vi "02_ui_plot_window.vi"() -> ()   [LabVIEW 2025]
uses:
  4c7a61b9-d50a-4fa5-8b88-644507a3af04.vi
  74ea501e-f43b-483f-8511-84a735437533.vi
  166e0385-1291-4ee6-a608-8b02bdaae3d2.vi
  b1158e5f-e22e-42fa-9d41-9ea4e4d0b9e3.vi
  31b119fa-27fe-4ebe-809c-2da1a8fd4d96.vi
  13143f16-a64c-4a8d-9511-2945b8db9dc5.vi
  9c1d92a2-1c85-4809-97a6-d36bf52cbad7.vi
  d684625a-03c4-4daf-8e9e-674a236ebb3e.vi
  fb960f78-e1fe-4b5d-8417-6d8be925c5cf.vi
  c135c75a-78bf-4448-8d92-d4bbbd51cd11.vi
  <vilib>/Utility/config.llb/Read Key (U32).vi
  <vilib>/Utility/config.llb/Read Key (Boolean).vi
  <vilib>/Utility/config.llb/Read Key (String).vi
  <vilib>/Utility/config.llb/Write Key (U32).vi
  <vilib>/Utility/config.llb/Write Key (Boolean).vi
  <vilib>/Utility/config.llb/Write Key (String).vi
  00_global_variables.vi
  <vilib>/Utility/config.llb/NI_LVConfig.lvlib
panel:
  out "loaded_config_path":path
  out "loaded_config_filename":string caption="Recent File"
  in  "open_config_plot_0":bool
  in  "safe_config_as_plot_0":bool
  in  "safe_config_plot_0":bool
  in  "select_plot_5":string(combo)="2"
  in  "select_plot_4":string(combo)="2"
  out "cursor_p5_1_prefix":string
  out "cursor_p4_1_prefix":string
  out "cursor_p5_2_prefix":string
  out "cursor_p4_2_prefix":string
  out "cursor_p5_2":dbl format="%#_6f"
  in  "color_picker_5":u32(colorbox)=14811391
  out "cursor_p5_1":dbl format="%#_6f"
  in  "enable_plot_5":bool caption="S11 - Imaginary"
  out "cursor_p4_2":dbl format="%#_6f"
  in  "color_picker_4":u32(colorbox)=49352
  out "cursor_p4_1":dbl format="%#_6f"
  in  "enable_plot_4":bool caption="S11 - Imaginary"
  in  "select_plot_3":string(combo)="2"
  in  "select_plot_2":string(combo)="2"
  in  "select_plot_1":string(combo)="2"
  in  "select_plot_0":string(combo)="2"
  out "cursor_p3_1_prefix":string
  out "cursor_p2_1_prefix":string
  out "cursor_p1_1_prefix":string
  out "cursor_p0_1_prefix":string
  out "cursor_p3_2_prefix":string
  out "cursor_p2_2_prefix":string
  out "cursor_p1_2_prefix":string
  out "cursor_p0_2_prefix":string
  out "cursor_p3_2":dbl format="%#_6f"
  in  "color_picker_3":u32(colorbox)=14468608
  out "cursor_p3_1":dbl format="%#_6f"
  in  "enable_plot_3":bool caption="S11 - Imaginary"
  out "cursor_p2_2":dbl format="%#_6f"
  in  "color_picker_2":u32(colorbox)=39219
  out "cursor_p2_1":dbl format="%#_6f"
  in  "enable_plot_2":bool caption="S11 - Imaginary"
  out "cursor_p1_2":dbl format="%#_6f"
  out "cursor_p0_2":dbl format="%#_6f"
  out "cursor_p0_freq_2":string caption="Frequenz"
  out "cursor_p0_wavel_2":dbl caption="Frequenz"
  out "cursor_p0_wavel_1":dbl caption="Frequenz"
  in  "color_picker_1":u32(colorbox)=14423100
  in  "color_picker_0":u32(colorbox)=26316
  out "cursor_p0_freq_1":string caption="Frequenz"
  out "cursor_p1_1":dbl format="%#_6f"
  out "cursor_p0_1":dbl format="%#_6f"
  in  "enable_plot_1":bool caption="S11 - Imaginary"
  in  "enable_plot_0":bool=TRUE
  out "plot_0":cluster{"array type (2D Dbl)":dbl[], dbl[]}[](graph)
  # "Cursor 2"
  # "Cursor 1"
  # "Hz"
  # "Frequency"
  # "Hz"
  # "Wavelength"
  # "m"
  # "m"
  # "Configuration"
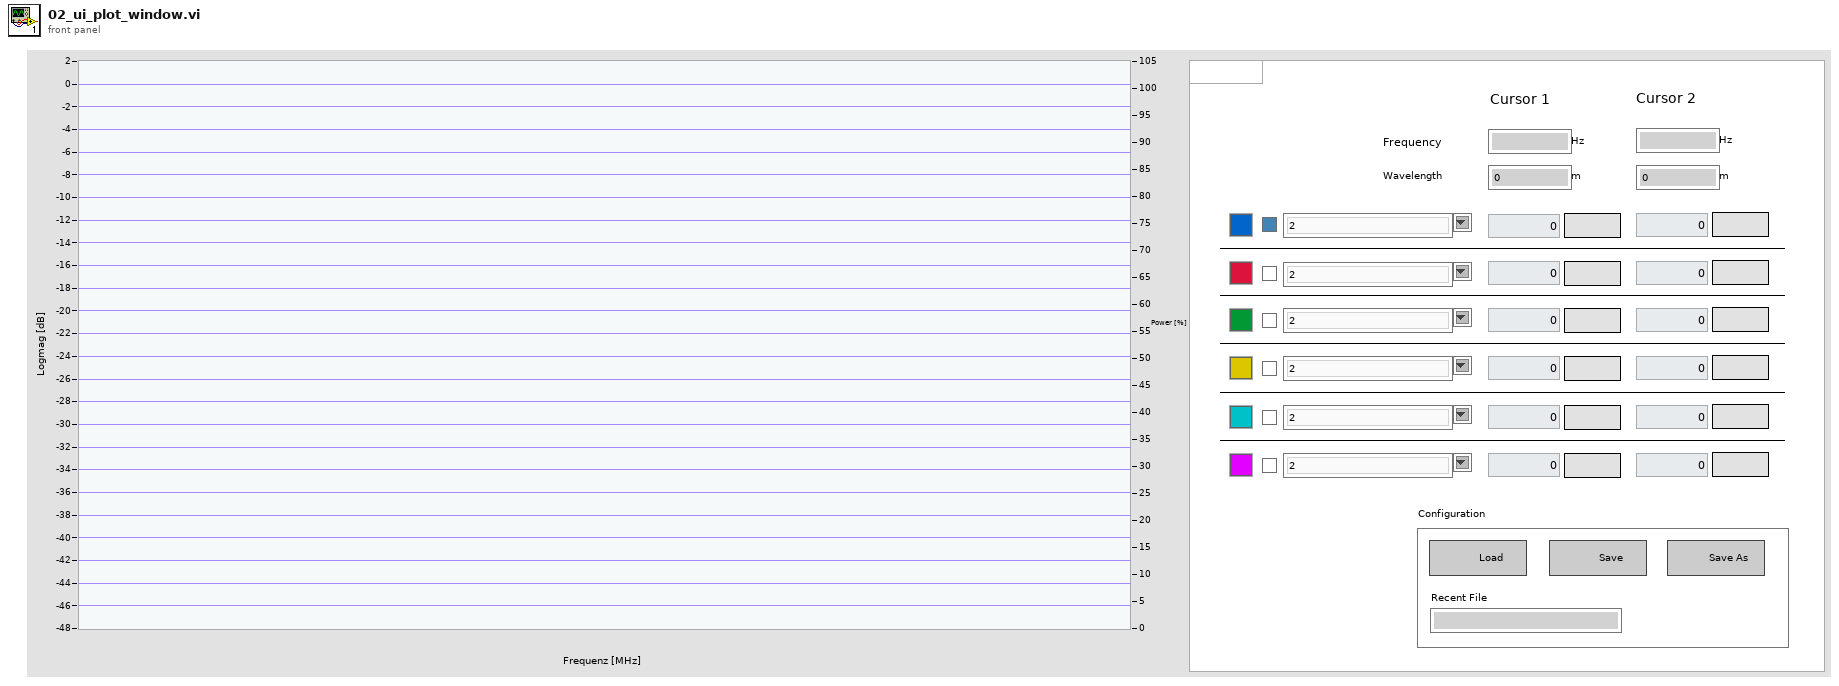
[diagram p1: front panel]
types:
  T1 = typedef "NI_LVConfig.lvlib/Config Data RefNum.ctl" = refnum<k1>
  T2 = typedef "LVComboBoxStrsAndValuesArrayTypeDef.ctl" = cluster{"String":string, "Value":string}[]
  T3 = cluster{"freq_array":dbl[], "data_array":dbl[]}[]
  T4 = cluster{"y_scale_id":u32, "unit":string, "prefix_enable":bool, "plot_id":u32}[]
  T5 = cluster{"y_scale_id":u32, "unit":string, "prefix_enable":bool, "plot_id":u32}
  T6 = typedef "LVCursorListTypeDef.ctl" = cluster{"Name":string, "Color":u32, "Style":u8, "Point Style":u8, "Name Visible":bool, "Allow Drag":bool, "Cursor Mode":u32, "Plot":i32, "Index":i32, "Position":cluster{"X":dbl, "Y":dbl}, "X Scale":u32, "Y Scale":u32, "Watch Plots":i32[], "Watch All Plots":bool, "Plot Area":i32, "Label Offset":cluster{"X":dbl, "Y":dbl}}[]
  T7 = cluster{"cursor_data":dbl[], "frequency":string, "wavelength_m":dbl}
  T8 = cluster{"cursor_0_color":u32, "cursor_1_color":u32}
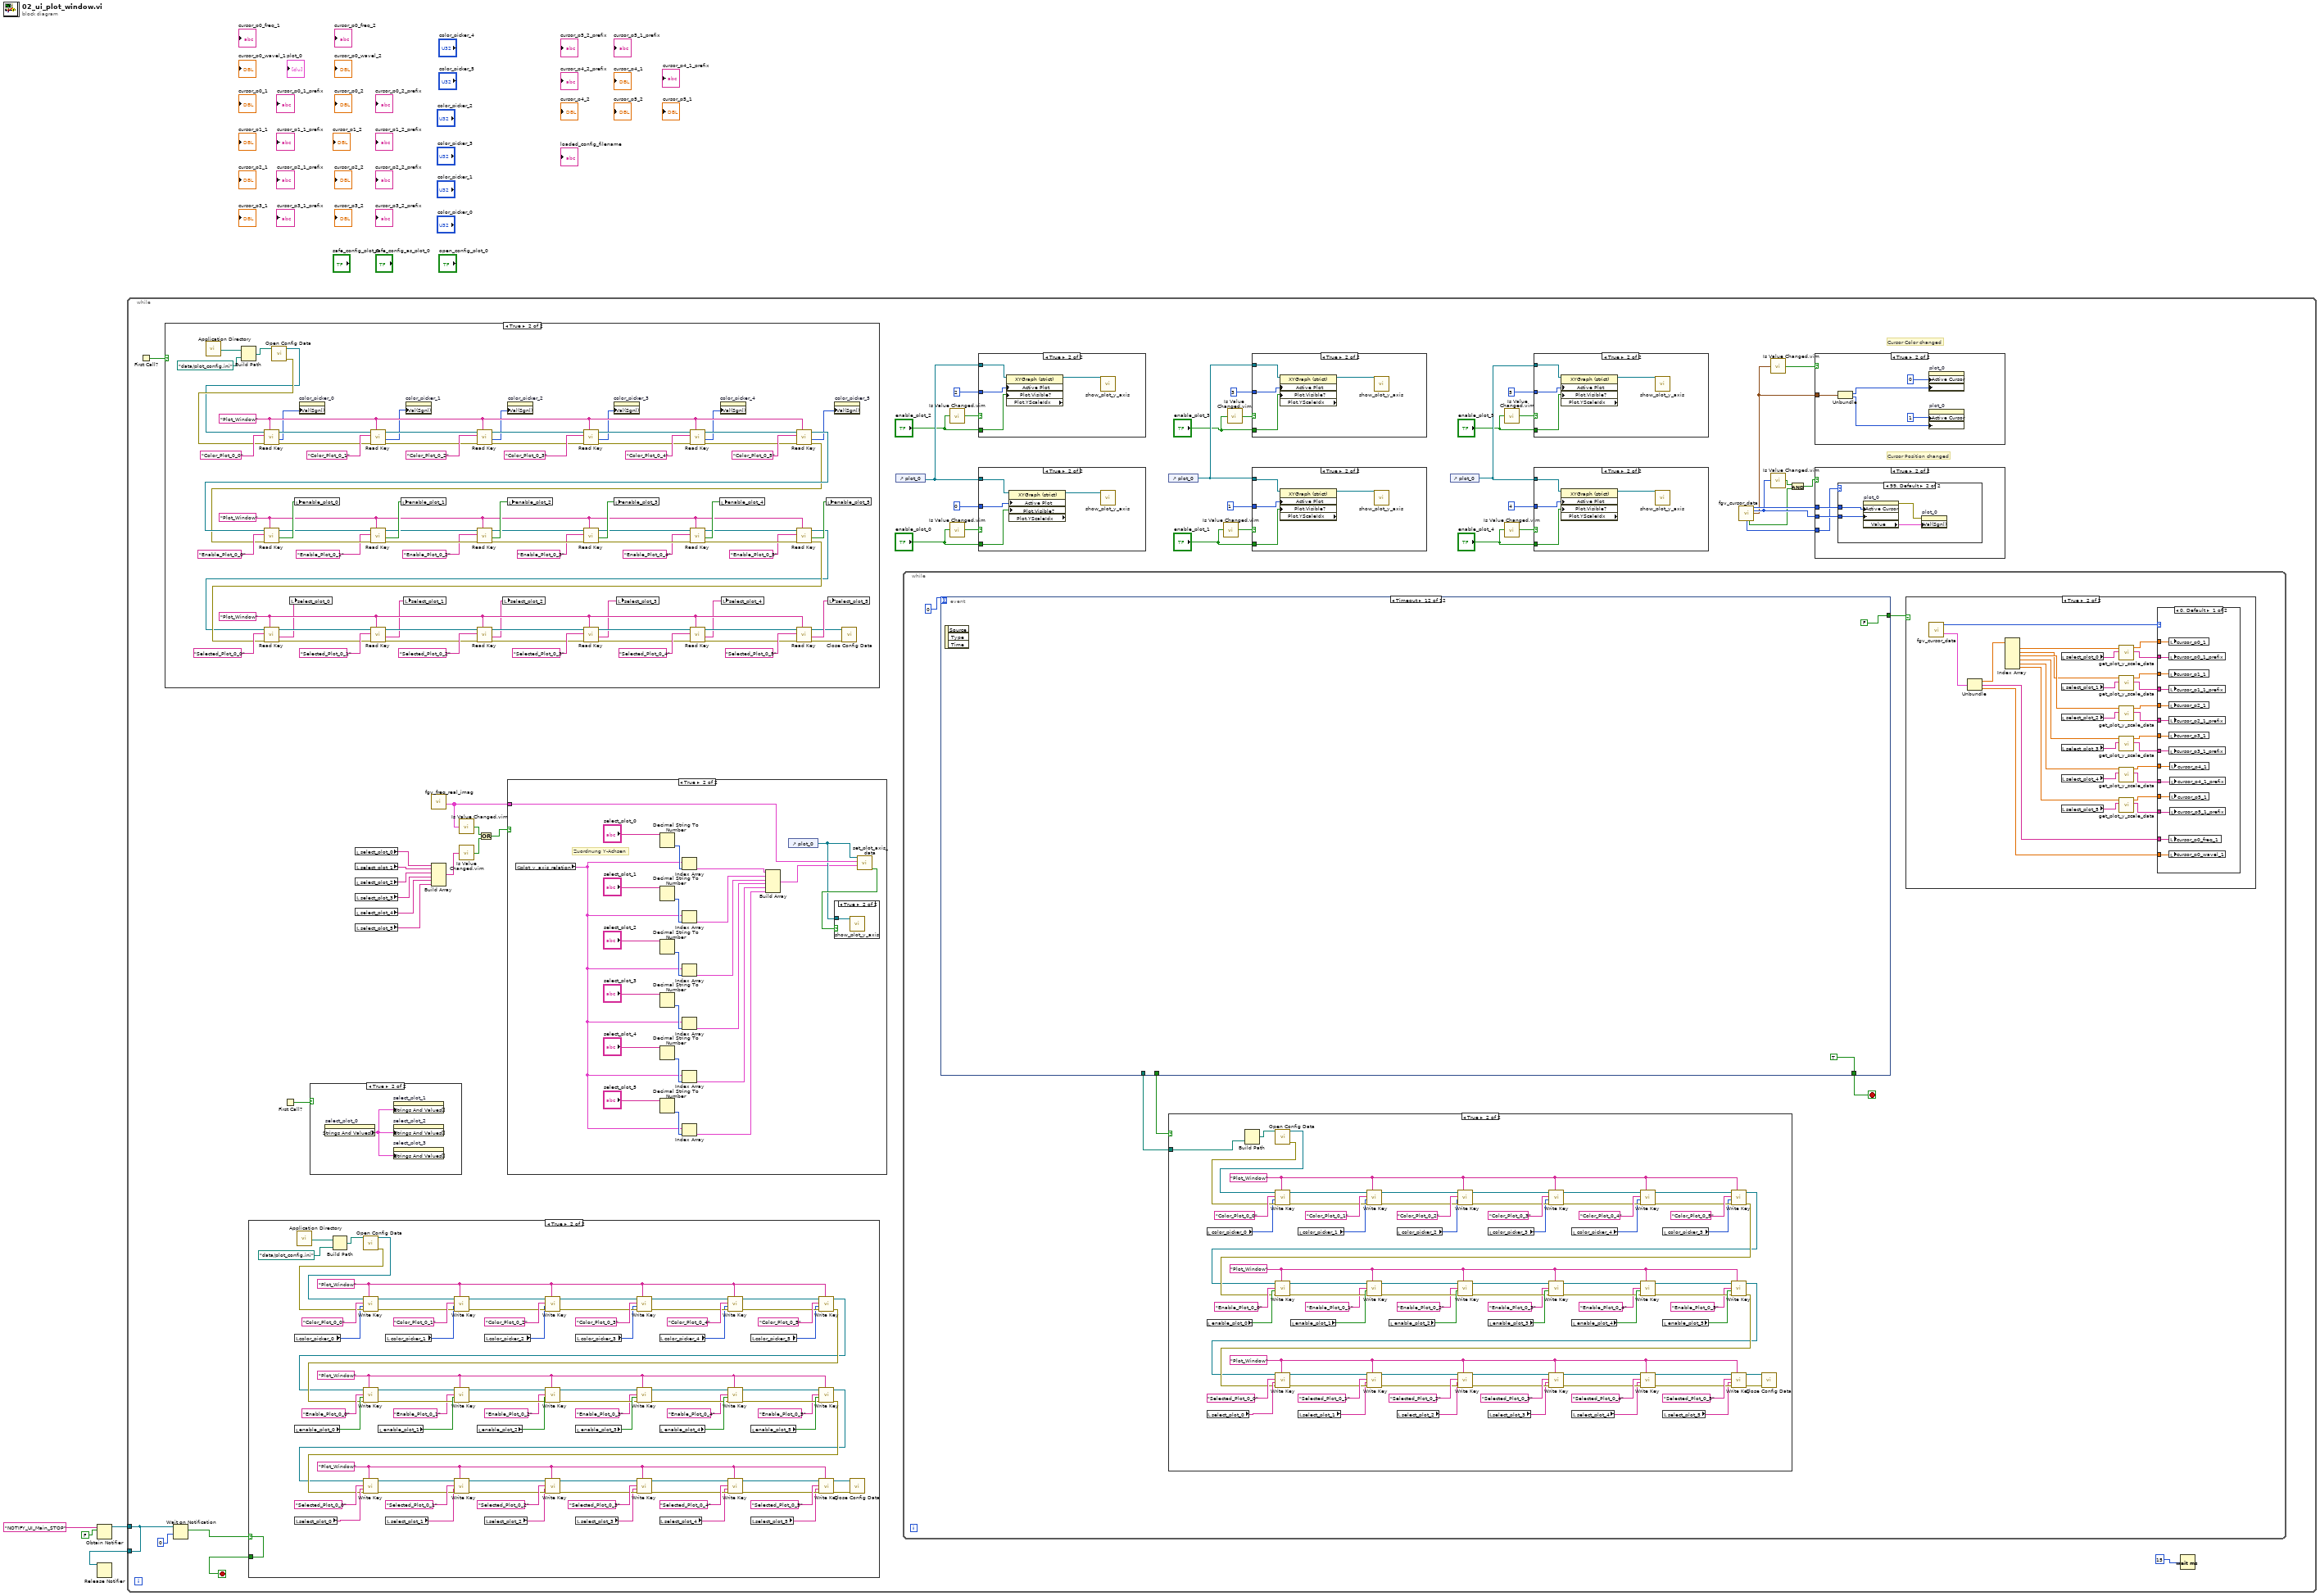
[diagram p0: block diagram]
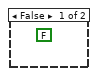
[diagram p11: hidden frame]
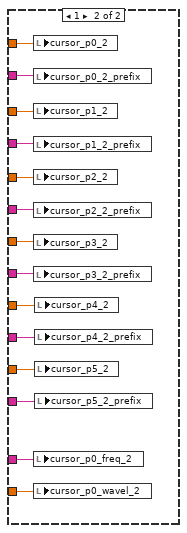
[diagram p18: hidden frame]
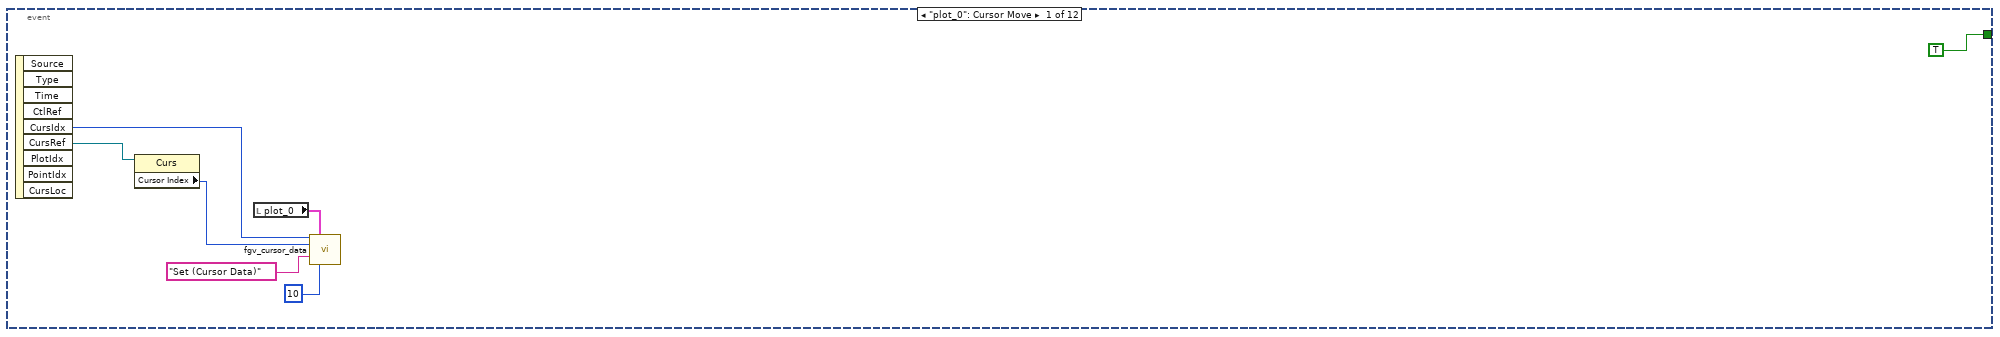
[diagram p19: hidden frame]
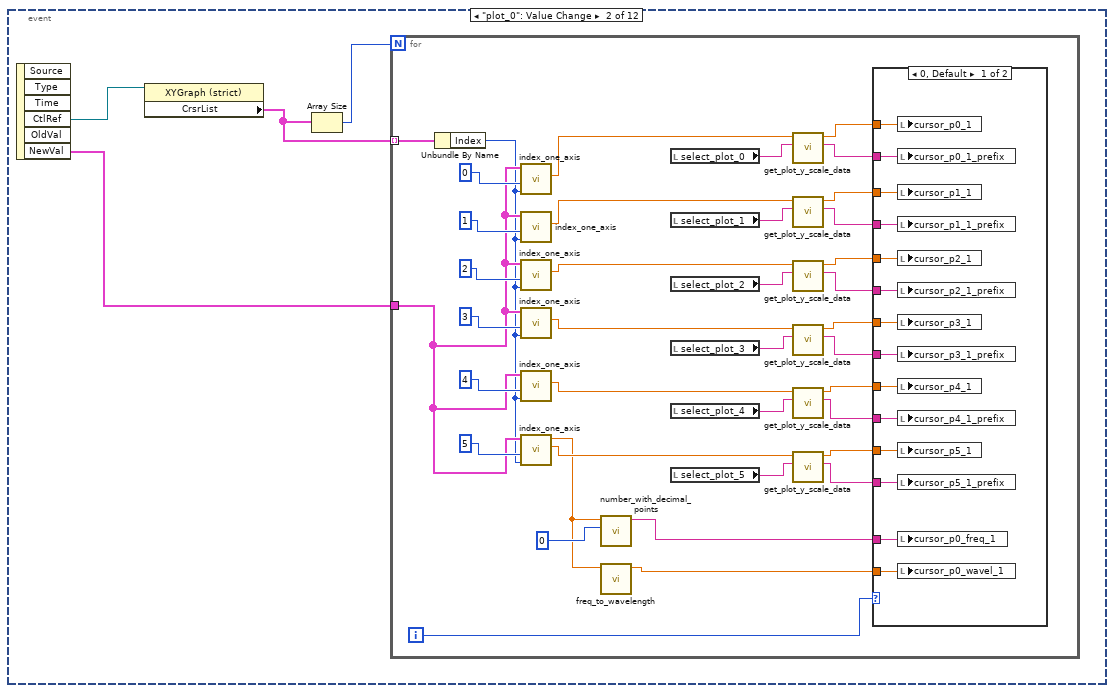
[diagram p20: hidden frame]
diagram:
  n1 = Obtain Notifier(name (unnamed)="NOTIFY_UI_Main_STOP", notification data type=FALSE) -> (notifier out=w2:refnum<notifier>)  [unwired: 2 in, 2 out]
  n2 = while {
    tunnel: w2 -> [w28]
    tunnel: [w28] -> w1
    stop <- w14 stop-if-true
    # "Cursor Color changed"
    # "Cursor Position changed"
    n3 = First Call?() -> (First Call?: T/F=w13:bool)
    n4 = case shown="True" w13 {
      frame False {
      }
      frame True {
        w166 = "Plot_Window" ("section")
        w201 = "Plot_Window" ("section")
        w208 = "Plot_Window" ("section")
        n5 = call <vilib>:"Application Directory.vi"() -> ("Application Directory"=w151:path)
        n6 = Build Path(base path=w151, name or relative path=path "data/plot_config.ini") -> (appended path=w157:path)
        n7 = call <vilib>:"Open Config Data.vi"("configuration file path"=w157) -> ("error out"=w155:errorcluster, "refnum"=w154:T1)  [unwired: 8 in, 1 out]
        n8 = call-poly <vilib>:"Read Key.vi"("section"=w208, "error in (no error)"=w155, "key"="Color_Plot_0_0", "refnum"=w154) -> ("error out"=w221:errorcluster, "value"=w150:u32, "refnum out"=w222:T1)  [unwired: 4 in, 1 out]
        n9 = property on="color_picker_0" class="ColBox"("Val(Sgnl)"=w150) -> ()  [unwired: 2 in, 2 out]
        n10 = call-poly <vilib>:"Read Key.vi"("section"=w208, "error in (no error)"=w221, "key"="Color_Plot_0_1", "refnum"=w222) -> ("error out"=w218:errorcluster, "value"=w149:u32, "refnum out"=w219:T1)  [unwired: 4 in, 1 out]
        n11 = property on="color_picker_1" class="ColBox"("Val(Sgnl)"=w149) -> ()  [unwired: 2 in, 2 out]
        n12 = call-poly <vilib>:"Read Key.vi"("section"=w208, "error in (no error)"=w218, "key"="Color_Plot_0_2", "refnum"=w219) -> ("error out"=w215:errorcluster, "value"=w145:u32, "refnum out"=w216:T1)  [unwired: 4 in, 1 out]
        n13 = property on="color_picker_2" class="ColBox"("Val(Sgnl)"=w145) -> ()  [unwired: 2 in, 2 out]
        n14 = call-poly <vilib>:"Read Key.vi"("section"=w208, "error in (no error)"=w215, "key"="Color_Plot_0_3", "refnum"=w216) -> ("error out"=w212:errorcluster, "value"=w146:u32, "refnum out"=w213:T1)  [unwired: 4 in, 1 out]
        n15 = property on="color_picker_3" class="ColBox"("Val(Sgnl)"=w146) -> ()  [unwired: 2 in, 2 out]
        n16 = call-poly <vilib>:"Read Key.vi"("section"=w208, "error in (no error)"=w212, "key"="Color_Plot_0_4", "refnum"=w213) -> ("error out"=w210:errorcluster, "value"=w147:u32, "refnum out"=w209:T1)  [unwired: 4 in, 1 out]
        n17 = property on="color_picker_4" class="ColBox"("Val(Sgnl)"=w147) -> ()  [unwired: 2 in, 2 out]
        n18 = call-poly <vilib>:"Read Key.vi"("section"=w208, "error in (no error)"=w210, "key"="Color_Plot_0_5", "refnum"=w209) -> ("error out"=w183:errorcluster, "value"=w148:u32, "refnum out"=w184:T1)  [unwired: 4 in, 1 out]
        n19 = call-poly <vilib>:"Read Key.vi"("section"=w201, "error in (no error)"=w183, "key"="Enable_Plot_0_0", "refnum"=w184) -> ("error out"=w188:errorcluster, "value"=w202:bool, "refnum out"=w187:T1)  [unwired: 4 in, 1 out]
        n20 = local write "enable_plot_0"(w202) -> ()
        n21 = call-poly <vilib>:"Read Key.vi"("section"=w201, "error in (no error)"=w188, "key"="Enable_Plot_0_1", "refnum"=w187) -> ("error out"=w191:errorcluster, "value"=w203:bool, "refnum out"=w190:T1)  [unwired: 4 in, 1 out]
        n22 = local write "enable_plot_1"(w203) -> ()
        n23 = call-poly <vilib>:"Read Key.vi"("section"=w201, "error in (no error)"=w191, "key"="Enable_Plot_0_2", "refnum"=w190) -> ("error out"=w194:errorcluster, "value"=w204:bool, "refnum out"=w193:T1)  [unwired: 4 in, 1 out]
        n24 = local write "enable_plot_2"(w204) -> ()
        n25 = call-poly <vilib>:"Read Key.vi"("section"=w201, "error in (no error)"=w194, "key"="Enable_Plot_0_3", "refnum"=w193) -> ("error out"=w197:errorcluster, "value"=w205:bool, "refnum out"=w196:T1)  [unwired: 4 in, 1 out]
        n26 = local write "enable_plot_3"(w205) -> ()
        n27 = call-poly <vilib>:"Read Key.vi"("section"=w201, "error in (no error)"=w197, "key"="Enable_Plot_0_4", "refnum"=w196) -> ("error out"=w199:errorcluster, "value"=w206:bool, "refnum out"=w200:T1)  [unwired: 4 in, 1 out]
        n28 = local write "enable_plot_4"(w206) -> ()
        n29 = call-poly <vilib>:"Read Key.vi"("section"=w201, "error in (no error)"=w199, "key"="Enable_Plot_0_5", "refnum"=w200) -> ("error out"=w159:errorcluster, "value"=w207:bool, "refnum out"=w158:T1)  [unwired: 4 in, 1 out]
        n30 = call-poly <vilib>:"Read Key.vi"("section"=w166, "error in (no error)"=w159, "key"="Selected_Plot_0_0", "refnum"=w158) -> ("error out"=w179:errorcluster, "value"=w165:string, "refnum out"=w180:T1)  [unwired: 4 in, 1 out]
        n31 = local write "select_plot_0"(w165) -> ()
        n32 = call-poly <vilib>:"Read Key.vi"("section"=w166, "error in (no error)"=w179, "key"="Selected_Plot_0_1", "refnum"=w180) -> ("error out"=w176:errorcluster, "value"=w164:string, "refnum out"=w177:T1)  [unwired: 4 in, 1 out]
        n33 = local write "select_plot_1"(w164) -> ()
        n34 = call-poly <vilib>:"Read Key.vi"("section"=w166, "error in (no error)"=w176, "key"="Selected_Plot_0_2", "refnum"=w177) -> ("error out"=w173:errorcluster, "value"=w163:string, "refnum out"=w174:T1)  [unwired: 4 in, 1 out]
        n35 = local write "select_plot_2"(w163) -> ()
        n36 = call-poly <vilib>:"Read Key.vi"("section"=w166, "error in (no error)"=w173, "key"="Selected_Plot_0_3", "refnum"=w174) -> ("error out"=w170:errorcluster, "value"=w162:string, "refnum out"=w171:T1)  [unwired: 4 in, 1 out]
        n37 = local write "select_plot_3"(w162) -> ()
        n38 = call-poly <vilib>:"Read Key.vi"("section"=w166, "error in (no error)"=w170, "key"="Selected_Plot_0_4", "refnum"=w171) -> ("error out"=w168:errorcluster, "value"=w161:string, "refnum out"=w167:T1)  [unwired: 4 in, 1 out]
        n39 = local write "select_plot_4"(w161) -> ()
        n40 = call-poly <vilib>:"Read Key.vi"("section"=w166, "error in (no error)"=w168, "key"="Selected_Plot_0_5", "refnum"=w167) -> ("error out"=w152:errorcluster, "value"=w160:string, "refnum out"=w153:T1)  [unwired: 4 in, 1 out]
        n41 = local write "enable_plot_5"(w207) -> ()
        n42 = local write "select_plot_5"(w160) -> ()
        n43 = property on="color_picker_5" class="ColBox"("Val(Sgnl)"=w148) -> ()  [unwired: 2 in, 2 out]
        n44 = call <vilib>:"Close Config Data.vi"("error in (no error)"=w152, "refnum"=w153) -> ()  [unwired: 8 in, 2 out]
      }
    }
    n45 = Wait on Notification(notifier=w28, timeout in ms (-1)=0) -> (notification=w15:bool)  [unwired: 2 in, 3 out]
    n46 = case shown="True" w15 {
      selector: w15 -> [_ w144]
      tunnel: [_ w144] -> w14
      frame False {
      }
      frame True {
        w71 = "Plot_Window" ("section")
        w116 = "Plot_Window" ("section")
        w65 = "Plot_Window" ("section")
        n47 = local read "color_picker_0"() -> (w123:u32)
        n48 = local read "enable_plot_0"() -> (w111:bool)
        n49 = local read "select_plot_0"() -> (w76:string)
        n50 = call <vilib>:"Application Directory.vi"() -> ("Application Directory"=w64:path)
        n51 = Build Path(base path=w64, name or relative path=path "data/plot_config.ini") -> (appended path=w130:path)
        n52 = call <vilib>:"Open Config Data.vi"("configuration file path"=w130) -> ("error out"=w128:errorcluster, "refnum"=w127:T1)  [unwired: 8 in, 1 out]
        n53 = call-poly <vilib>:"Write Key.vi"("section"=w65, "error in (no error)"=w128, "value"=w123, "key"="Color_Plot_0_0", "refnum"=w127) -> ("error out"=w140:errorcluster, "refnum out"=w141:T1)  [unwired: 4 in, 1 out]
        n54 = local read "enable_plot_1"() -> (w112:bool)
        n55 = local read "color_picker_1"() -> (w122:u32)
        n56 = local read "select_plot_1"() -> (w75:string)
        n57 = call-poly <vilib>:"Write Key.vi"("section"=w65, "error in (no error)"=w140, "value"=w122, "key"="Color_Plot_0_1", "refnum"=w141) -> ("error out"=w137:errorcluster, "refnum out"=w138:T1)  [unwired: 4 in, 1 out]
        n58 = local read "enable_plot_2"() -> (w113:bool)
        n59 = local read "color_picker_2"() -> (w121:u32)
        n60 = local read "select_plot_2"() -> (w74:string)
        n61 = call-poly <vilib>:"Write Key.vi"("section"=w65, "error in (no error)"=w137, "value"=w121, "key"="Color_Plot_0_2", "refnum"=w138) -> ("error out"=w134:errorcluster, "refnum out"=w135:T1)  [unwired: 4 in, 1 out]
        n62 = local read "color_picker_3"() -> (w118:u32)
        n63 = local read "enable_plot_3"() -> (w117:bool)
        n64 = local read "select_plot_3"() -> (w70:string)
        n65 = call-poly <vilib>:"Write Key.vi"("section"=w65, "error in (no error)"=w134, "value"=w118, "key"="Color_Plot_0_3", "refnum"=w135) -> ("error out"=w131:errorcluster, "refnum out"=w132:T1)  [unwired: 4 in, 1 out]
        n66 = local read "color_picker_4"() -> (w120:u32)
        n67 = local read "enable_plot_4"() -> (w114:bool)
        n68 = local read "select_plot_4"() -> (w73:string)
        n69 = call-poly <vilib>:"Write Key.vi"("section"=w65, "error in (no error)"=w131, "value"=w120, "key"="Color_Plot_0_4", "refnum"=w132) -> ("error out"=w124:errorcluster, "refnum out"=w125:T1)  [unwired: 4 in, 1 out]
        n70 = local read "color_picker_5"() -> (w119:u32)
        n71 = local read "enable_plot_5"() -> (w115:bool)
        n72 = local read "select_plot_5"() -> (w72:string)
        n73 = call-poly <vilib>:"Write Key.vi"("section"=w65, "error in (no error)"=w124, "value"=w119, "key"="Color_Plot_0_5", "refnum"=w125) -> ("error out"=w94:errorcluster, "refnum out"=w93:T1)  [unwired: 4 in, 1 out]
        n74 = call-poly <vilib>:"Write Key.vi"("section"=w116, "error in (no error)"=w94, "value"=w111, "key"="Enable_Plot_0_0", "refnum"=w93) -> ("error out"=w98:errorcluster, "refnum out"=w97:T1)  [unwired: 4 in, 1 out]
        n75 = call-poly <vilib>:"Write Key.vi"("section"=w116, "error in (no error)"=w98, "value"=w112, "key"="Enable_Plot_0_1", "refnum"=w97) -> ("error out"=w101:errorcluster, "refnum out"=w100:T1)  [unwired: 4 in, 1 out]
        n76 = call-poly <vilib>:"Write Key.vi"("section"=w116, "error in (no error)"=w101, "value"=w113, "key"="Enable_Plot_0_2", "refnum"=w100) -> ("error out"=w104:errorcluster, "refnum out"=w103:T1)  [unwired: 4 in, 1 out]
        n77 = call-poly <vilib>:"Write Key.vi"("section"=w116, "error in (no error)"=w104, "value"=w117, "key"="Enable_Plot_0_3", "refnum"=w103) -> ("error out"=w107:errorcluster, "refnum out"=w106:T1)  [unwired: 4 in, 1 out]
        n78 = call-poly <vilib>:"Write Key.vi"("section"=w116, "error in (no error)"=w107, "value"=w114, "key"="Enable_Plot_0_4", "refnum"=w106) -> ("error out"=w110:errorcluster, "refnum out"=w109:T1)  [unwired: 4 in, 1 out]
        n79 = call-poly <vilib>:"Write Key.vi"("section"=w116, "error in (no error)"=w110, "value"=w115, "key"="Enable_Plot_0_5", "refnum"=w109) -> ("error out"=w69:errorcluster, "refnum out"=w68:T1)  [unwired: 4 in, 1 out]
        n80 = call-poly <vilib>:"Write Key.vi"("section"=w71, "error in (no error)"=w69, "value"=w76, "key"="Selected_Plot_0_0", "refnum"=w68) -> ("error out"=w89:errorcluster, "refnum out"=w90:T1)  [unwired: 4 in, 1 out]
        n81 = call-poly <vilib>:"Write Key.vi"("section"=w71, "error in (no error)"=w89, "value"=w75, "key"="Selected_Plot_0_1", "refnum"=w90) -> ("error out"=w86:errorcluster, "refnum out"=w87:T1)  [unwired: 4 in, 1 out]
        n82 = call-poly <vilib>:"Write Key.vi"("section"=w71, "error in (no error)"=w86, "value"=w74, "key"="Selected_Plot_0_2", "refnum"=w87) -> ("error out"=w83:errorcluster, "refnum out"=w84:T1)  [unwired: 4 in, 1 out]
        n83 = call-poly <vilib>:"Write Key.vi"("section"=w71, "error in (no error)"=w83, "value"=w70, "key"="Selected_Plot_0_3", "refnum"=w84) -> ("error out"=w80:errorcluster, "refnum out"=w81:T1)  [unwired: 4 in, 1 out]
        n84 = call-poly <vilib>:"Write Key.vi"("section"=w71, "error in (no error)"=w80, "value"=w73, "key"="Selected_Plot_0_4", "refnum"=w81) -> ("error out"=w77:errorcluster, "refnum out"=w78:T1)  [unwired: 4 in, 1 out]
        n85 = call-poly <vilib>:"Write Key.vi"("section"=w71, "error in (no error)"=w77, "value"=w72, "key"="Selected_Plot_0_5", "refnum"=w78) -> ("error out"=w66:errorcluster, "refnum out"=w67:T1)  [unwired: 4 in, 1 out]
        n86 = call <vilib>:"Close Config Data.vi"("error in (no error)"=w66, "refnum"=w67) -> ()  [unwired: 8 in, 2 out]
      }
    }
    n87 = First Call?() -> (First Call?: T/F=w25:bool)
    n88 = case shown="True" w25 {
      frame False {
      }
      frame True {
        n89 = property on="select_plot_0" class="CmbBox"() -> ("Strings And Values[]"=w233:T2)  [unwired: 2 in, 2 out]
        n90 = property on="select_plot_1" class="CmbBox"("Strings And Values[]"=w233) -> ()  [unwired: 2 in, 2 out]
        n91 = property on="select_plot_2" class="CmbBox"("Strings And Values[]"=w233) -> ()  [unwired: 2 in, 2 out]
        n92 = property on="select_plot_3" class="CmbBox"("Strings And Values[]"=w233) -> ()  [unwired: 2 in, 2 out]
      }
    }
    n93 = local read "select_plot_0"() -> (w40:string)
    n94 = local read "select_plot_1"() -> (w39:string)
    n95 = local read "select_plot_2"() -> (w38:string)
    n96 = local read "select_plot_3"() -> (w37:string)
    n97 = local read "select_plot_4"() -> (w17:string)
    n98 = local read "select_plot_5"() -> (w16:string)
    n99 = call "fgv_freq_real_imag.vi"() -> ("plot_data"=w26:T3)  [unwired: 8 in, 3 out]
    n100 = Build Array(w40, w39, w38, w37, w17, w16) -> (w36:string[])
    n101 = call "Is Value Changed.vim"("value"=w26) -> ("changed or first call?"=w41:bool)
    n102 = call "Is Value Changed.vim"("value"=w36) -> ("changed or first call?"=w35:bool)
    n103 = Or(x=w41, y=w35) -> (x .or. y?=w42:bool)
    n104 = case shown="True" w42 {
      tunnel: w26 -> [_ w252]
      frame False {
        (unwired) FALSE
      }
      frame True {
        # "Zuordnung Y-Achsen"
        n105 = global read "00_global_variables.vi" "plot_y_axis_relation"() -> (w240:T4)
        n106 = Decimal String To Number(string="select_plot_0") -> (number=w256:i32)  [unwired: 2 in, 1 out]
        n107 = Decimal String To Number(string="select_plot_1") -> (number=w255:i32)  [unwired: 2 in, 1 out]
        n108 = Decimal String To Number(string="select_plot_2") -> (number=w254:i32)  [unwired: 2 in, 1 out]
        n109 = Decimal String To Number(string="select_plot_3") -> (number=w253:i32)  [unwired: 2 in, 1 out]
        n110 = Decimal String To Number(string="select_plot_4") -> (number=w244:i32)  [unwired: 2 in, 1 out]
        n111 = Decimal String To Number(string="select_plot_5") -> (number=w243:i32)  [unwired: 2 in, 1 out]
        n112 = Index Array(array=w240, index=w256) -> (element=w249:T5)
        n113 = Index Array(array=w240, index=w255) -> (element=w248:T5)
        n114 = Index Array(array=w240, index=w254) -> (element=w247:T5)
        n115 = Index Array(array=w240, index=w253) -> (element=w246:T5)
        n116 = Index Array(array=w240, index=w244) -> (element=w239:T5)
        n117 = Index Array(array=w240, index=w243) -> (element=w238:T5)
        n118 = Build Array(w249, w248, w247, w246, w239, w238) -> (w245:T4)
        n119 = control-ref of="plot_0"() -> (w250:refnum<vi>)
        n120 = call "set_plot_axis_data.vi"("plot_allocation"=w245, "plot_data"=w252, "reference"=w250) -> ("done"=w251:bool)  [unwired: 8 in]
        n121 = case shown="True" w251 {
          tunnel: w250 -> [_ w261]
          frame False {
          }
          frame True {
            n122 = call "show_plot_y_axis.vi"("plot_ref_in"=w261) -> ()  [unwired: 9 in, 2 out]
          }
        }
      }
    }
    n123 = control-ref of="plot_0"() -> (w44:refnum<vi>)
    n124 = while {
      stop <- w278 stop-if-true
      n125 = event shown="[11] Timeout" {
        selector: _ -> [_ _ _ _ _ _ _ _ _ _ _ _]
        dyn-events: _ -> [_ _ _ _ _ _ _ _ _ _ _ _]
        timeout: 0 -> [_ _ _ _ _ _ _ _ _ _ _ _]
        tunnel: [_ _ _ _ _ _ _ _ _ _ _ TRUE] -> w278
        tunnel: [TRUE _ _ _ _ _ _ _ _ _ _ FALSE] -> w276
        tunnel: [_ _ _ _ _ _ _ _ _ w594 w616 _] -> w275
        tunnel: [_ _ _ _ _ _ _ _ _ w593 w615 _] -> w274
        event "plot_0": Cursor Move {
          n126 = event-data() -> ("CursIdx"=w421:i32, "CursRef"=w417:refnum<vi>)  [unwired: 1 in, 7 out]
          n127 = property on="Property Node" class="Curs"(reference=w417) -> ("Cursor Index"=w416:i32)  [unwired: 1 in, 2 out]
          n128 = local read "plot_0"() -> (w419:cluster{"array type (2D Dbl)":dbl[], dbl[]}[])
          n129 = call "fgv_cursor_data.vi"("cursor_idx_set"=w421, "plot_data_set"=w419, "cursor_pos_set"=w416, "mode"="Set (Cursor Data)", "plot_id_set"=10) -> ()  [unwired: 4 in, 7 out]
        }
        event "plot_0": Value Change {
          n130 = event-data() -> ("CtlRef"=w423:refnum<vi>, "NewVal"=w422:cluster{"array type (2D Dbl)":dbl[], dbl[]}[])  [unwired: 1 in, 4 out]
          n131 = property on="Property Node" class="XYGraph (strict)"(reference=w423) -> ("CrsrList"=w425:T6)  [unwired: 1 in, 2 out]
          n132 = Array Size(array=w425) -> (size(s)=w424:i32)
          n133 = for {
            N: w424 -> [_]
            tunnel: w425 -> [w463] mode=indexing
            tunnel: w422 -> [w432]
            i -> [w445]
            n134 = Unbundle By Name(w463) -> ("Index"=w431:i32)
            n135 = call "index_one_axis.vi"("x_index"=w431, "curve_sel"=0 ("x_index"), "graph_data"=w432) -> ("Y"=w442:dbl)  [unwired: 7 in, 1 out]
            n136 = call "index_one_axis.vi"("x_index"=w431, "curve_sel"=1 ("x_index"), "graph_data"=w432) -> ("Y"=w441:dbl)  [unwired: 7 in, 1 out]
            n137 = call "index_one_axis.vi"("x_index"=w431, "curve_sel"=2 ("x_index"), "graph_data"=w432) -> ("Y"=w440:dbl)  [unwired: 7 in, 1 out]
            n138 = call "index_one_axis.vi"("x_index"=w431, "curve_sel"=3 ("x_index"), "graph_data"=w432) -> ("Y"=w439:dbl)  [unwired: 7 in, 1 out]
            n139 = call "index_one_axis.vi"("x_index"=w431, "curve_sel"=4 ("x_index"), "graph_data"=w432) -> ("Y"=w438:dbl)  [unwired: 7 in, 1 out]
            n140 = call "index_one_axis.vi"("x_index"=w431, "curve_sel"=5 ("x_index"), "graph_data"=w432) -> ("Y"=w433:dbl, "X"=w430:dbl)  [unwired: 7 in]
            n141 = call "number_with_decimal_points.vi"("Precision"=i16 0, "Double"=w430) -> ("String"=w443:string)  [unwired: 5 in]
            n142 = call "freq_to_wavelength.vi"("frequency_hz"=w430) -> ("wavelength_m"=w444:dbl)  [unwired: 10 in]
            n143 = local read "select_plot_0"() -> (w457:string)
            n144 = local read "select_plot_1"() -> (w456:string)
            n145 = local read "select_plot_2"() -> (w455:string)
            n146 = local read "select_plot_3"() -> (w448:string)
            n147 = local read "select_plot_4"() -> (w437:string)
            n148 = local read "select_plot_5"() -> (w434:string)
            n149 = call "get_plot_y_scale_data.vi"("plot_selector"=w457, "cursor_value_in"=w442) -> ("prefix/unit"=w452:string, "cursor_value_out"=w451:dbl)  [unwired: 8 in]
            n150 = call "get_plot_y_scale_data.vi"("plot_selector"=w456, "cursor_value_in"=w441) -> ("prefix/unit"=w453:string, "cursor_value_out"=w450:dbl)  [unwired: 8 in]
            n151 = call "get_plot_y_scale_data.vi"("plot_selector"=w455, "cursor_value_in"=w440) -> ("prefix/unit"=w454:string, "cursor_value_out"=w449:dbl)  [unwired: 8 in]
            n152 = call "get_plot_y_scale_data.vi"("plot_selector"=w448, "cursor_value_in"=w439) -> ("prefix/unit"=w446:string, "cursor_value_out"=w447:dbl)  [unwired: 8 in]
            n153 = call "get_plot_y_scale_data.vi"("plot_selector"=w437, "cursor_value_in"=w438) -> ("prefix/unit"=w427:string, "cursor_value_out"=w426:dbl)  [unwired: 8 in]
            n154 = call "get_plot_y_scale_data.vi"("plot_selector"=w434, "cursor_value_in"=w433) -> ("prefix/unit"=w429:string, "cursor_value_out"=w428:dbl)  [unwired: 8 in]
            n155 = case shown="0, Default" w445 {
              tunnel: w451 -> [w477 w491]
              tunnel: w450 -> [w476 w490]
              tunnel: w449 -> [w475 w489]
              tunnel: w447 -> [w474 w488]
              tunnel: w443 -> [w473 w487]
              tunnel: w444 -> [w472 w486]
              tunnel: w446 -> [w471 w482]
              tunnel: w452 -> [w470 w485]
              tunnel: w453 -> [w469 w484]
              tunnel: w454 -> [w468 w483]
              tunnel: w429 -> [w467 w478]
              tunnel: w428 -> [w466 w479]
              tunnel: w427 -> [w465 w480]
              tunnel: w426 -> [w464 w481]
              frame 0, Default {
                n156 = local write "cursor_p0_1"(w477) -> ()
                n157 = local write "cursor_p0_1_prefix"(w470) -> ()
                n158 = local write "cursor_p1_1"(w476) -> ()
                n159 = local write "cursor_p1_1_prefix"(w469) -> ()
                n160 = local write "cursor_p2_1"(w475) -> ()
                n161 = local write "cursor_p2_1_prefix"(w468) -> ()
                n162 = local write "cursor_p3_1"(w474) -> ()
                n163 = local write "cursor_p3_1_prefix"(w471) -> ()
                n164 = local write "cursor_p4_1"(w464) -> ()
                n165 = local write "cursor_p4_1_prefix"(w465) -> ()
                n166 = local write "cursor_p5_1"(w466) -> ()
                n167 = local write "cursor_p5_1_prefix"(w467) -> ()
                n168 = local write "cursor_p0_freq_1"(w473) -> ()
                n169 = local write "cursor_p0_wavel_1"(w472) -> ()
              }
              frame 1 {
                n170 = local write "cursor_p0_2"(w491) -> ()
                n171 = local write "cursor_p0_2_prefix"(w485) -> ()
                n172 = local write "cursor_p1_2"(w490) -> ()
                n173 = local write "cursor_p1_2_prefix"(w484) -> ()
                n174 = local write "cursor_p2_2"(w489) -> ()
                n175 = local write "cursor_p2_2_prefix"(w483) -> ()
                n176 = local write "cursor_p3_2"(w488) -> ()
                n177 = local write "cursor_p3_2_prefix"(w482) -> ()
                n178 = local write "cursor_p4_2"(w481) -> ()
                n179 = local write "cursor_p4_2_prefix"(w480) -> ()
                n180 = local write "cursor_p5_2"(w479) -> ()
                n181 = local write "cursor_p5_2_prefix"(w478) -> ()
                n182 = local write "cursor_p0_freq_2"(w487) -> ()
                n183 = local write "cursor_p0_wavel_2"(w486) -> ()
              }
            }
          }
        }
        event "color_picker_0": Value Change {
          n184 = event-data() -> ("NewVal"=w492:u32)  [unwired: 1 in, 5 out]
          n185 = property on="plot_0" class="XYGraph (strict)"("Active Plot"=u32 0, "Plot.Plot Color"=w492) -> ()  [unwired: 2 in, 2 out]
        }
        event "color_picker_1": Value Change {
          n186 = event-data() -> ("NewVal"=w494:u32)  [unwired: 1 in, 5 out]
          n187 = property on="plot_0" class="XYGraph (strict)"("Active Plot"=u32 1, "Plot.Plot Color"=w494) -> ()  [unwired: 2 in, 2 out]
        }
        event "color_picker_2": Value Change {
          n188 = event-data() -> ("NewVal"=w496:u32)  [unwired: 1 in, 5 out]
          n189 = property on="plot_0" class="XYGraph (strict)"("Active Plot"=u32 2, "Plot.Plot Color"=w496) -> ()  [unwired: 2 in, 2 out]
        }
        event "color_picker_3": Value Change {
          n190 = event-data() -> ("NewVal"=w498:u32)  [unwired: 1 in, 5 out]
          n191 = property on="plot_0" class="XYGraph (strict)"("Active Plot"=u32 3, "Plot.Plot Color"=w498) -> ()  [unwired: 2 in, 2 out]
        }
        event "color_picker_4": Value Change {
          n192 = event-data() -> ("NewVal"=w500:u32)  [unwired: 1 in, 5 out]
          n193 = property on="plot_0" class="XYGraph (strict)"("Active Plot"=u32 4, "Plot.Plot Color"=w500) -> ()  [unwired: 2 in, 2 out]
        }
        event "color_picker_5": Value Change {
          n194 = event-data() -> ("NewVal"=w502:u32)  [unwired: 1 in, 5 out]
          n195 = property on="plot_0" class="XYGraph (strict)"("Active Plot"=u32 5, "Plot.Plot Color"=w502) -> ()  [unwired: 2 in, 2 out]
        }
        event "open_config_plot_0": Value Change {
          n196 = event-data() -> ("NewVal"=w504:bool)  [unwired: 1 in, 5 out]
          n197 = case shown="True" w504 {
            selector: w504 -> [_ w507]
            frame False {
            }
            frame True {
              n198 = Not(x=w507) -> (.not. x?=w506:bool)
              n199 = call "File Dialog2"("pattern (all files)"="*.ini" ("pattern label"), "pattern label"="INI-File") -> ("selected path"=w508:path, "cancelled"=w512:bool, "error out"=w505:errorcluster)  [unwired: 10 in, 1 out]
              n200 = local write "open_config_plot_0"(w506) -> ()
              n201 = Not(x=w512) -> (.not. x?=w509:bool)
              n202 = call <vilib>:"Clear Errors.vi"("error in (no error)"=w505) -> ()  [unwired: 5 in, 2 out]
              n203 = case shown="True" w509 {
                tunnel: w508 -> [_ w513]
                frame False {
                }
                frame True {
                  w534 = "Plot_Window" ("section")
                  w569 = "Plot_Window" ("section")
                  w576 = "Plot_Window" ("section")
                  n204 = Build Path(name or relative path=w513) -> (appended path=w525:path)  [unwired: 1 in]
                  n205 = call <vilib>:"Open Config Data.vi"("configuration file path"=w525) -> ("error out"=w524:errorcluster, "refnum"=w523:T1)  [unwired: 8 in, 1 out]
                  n206 = call-poly <vilib>:"Read Key.vi"("section"=w576, "error in (no error)"=w524, "key"="Color_Plot_0_0", "refnum"=w523) -> ("error out"=w589:errorcluster, "value"=w520:u32, "refnum out"=w590:T1)  [unwired: 4 in, 1 out]
                  n207 = property on="color_picker_0" class="ColBox"("Val(Sgnl)"=w520) -> ()  [unwired: 2 in, 2 out]
                  n208 = Strip Path(path=w513) -> (name=w514:string)  [unwired: 1 out]
                  n209 = local write "loaded_config_filename"(w514) -> ()
                  n210 = call-poly <vilib>:"Read Key.vi"("section"=w576, "error in (no error)"=w589, "key"="Color_Plot_0_1", "refnum"=w590) -> ("error out"=w586:errorcluster, "value"=w519:u32, "refnum out"=w587:T1)  [unwired: 4 in, 1 out]
                  n211 = property on="color_picker_1" class="ColBox"("Val(Sgnl)"=w519) -> ()  [unwired: 2 in, 2 out]
                  n212 = call-poly <vilib>:"Read Key.vi"("section"=w576, "error in (no error)"=w586, "key"="Color_Plot_0_2", "refnum"=w587) -> ("error out"=w583:errorcluster, "value"=w518:u32, "refnum out"=w584:T1)  [unwired: 4 in, 1 out]
                  n213 = property on="color_picker_2" class="ColBox"("Val(Sgnl)"=w518) -> ()  [unwired: 2 in, 2 out]
                  n214 = call-poly <vilib>:"Read Key.vi"("section"=w576, "error in (no error)"=w583, "key"="Color_Plot_0_3", "refnum"=w584) -> ("error out"=w580:errorcluster, "value"=w517:u32, "refnum out"=w581:T1)  [unwired: 4 in, 1 out]
                  n215 = property on="color_picker_3" class="ColBox"("Val(Sgnl)"=w517) -> ()  [unwired: 2 in, 2 out]
                  n216 = call-poly <vilib>:"Read Key.vi"("section"=w576, "error in (no error)"=w580, "key"="Color_Plot_0_4", "refnum"=w581) -> ("error out"=w578:errorcluster, "value"=w516:u32, "refnum out"=w577:T1)  [unwired: 4 in, 1 out]
                  n217 = property on="color_picker_4" class="ColBox"("Val(Sgnl)"=w516) -> ()  [unwired: 2 in, 2 out]
                  n218 = call-poly <vilib>:"Read Key.vi"("section"=w576, "error in (no error)"=w578, "key"="Color_Plot_0_5", "refnum"=w577) -> ("error out"=w551:errorcluster, "value"=w515:u32, "refnum out"=w552:T1)  [unwired: 4 in, 1 out]
                  n219 = call-poly <vilib>:"Read Key.vi"("section"=w569, "error in (no error)"=w551, "key"="Enable_Plot_0_0", "refnum"=w552) -> ("error out"=w556:errorcluster, "value"=w570:bool, "refnum out"=w555:T1)  [unwired: 4 in, 1 out]
                  n220 = local write "enable_plot_0"(w570) -> ()
                  n221 = call-poly <vilib>:"Read Key.vi"("section"=w569, "error in (no error)"=w556, "key"="Enable_Plot_0_1", "refnum"=w555) -> ("error out"=w559:errorcluster, "value"=w571:bool, "refnum out"=w558:T1)  [unwired: 4 in, 1 out]
                  n222 = local write "enable_plot_1"(w571) -> ()
                  n223 = call-poly <vilib>:"Read Key.vi"("section"=w569, "error in (no error)"=w559, "key"="Enable_Plot_0_2", "refnum"=w558) -> ("error out"=w562:errorcluster, "value"=w572:bool, "refnum out"=w561:T1)  [unwired: 4 in, 1 out]
                  n224 = local write "enable_plot_2"(w572) -> ()
                  n225 = call-poly <vilib>:"Read Key.vi"("section"=w569, "error in (no error)"=w562, "key"="Enable_Plot_0_3", "refnum"=w561) -> ("error out"=w565:errorcluster, "value"=w573:bool, "refnum out"=w564:T1)  [unwired: 4 in, 1 out]
                  n226 = local write "enable_plot_3"(w573) -> ()
                  n227 = call-poly <vilib>:"Read Key.vi"("section"=w569, "error in (no error)"=w565, "key"="Enable_Plot_0_4", "refnum"=w564) -> ("error out"=w567:errorcluster, "value"=w574:bool, "refnum out"=w568:T1)  [unwired: 4 in, 1 out]
                  n228 = local write "enable_plot_4"(w574) -> ()
                  n229 = call-poly <vilib>:"Read Key.vi"("section"=w569, "error in (no error)"=w567, "key"="Enable_Plot_0_5", "refnum"=w568) -> ("error out"=w527:errorcluster, "value"=w575:bool, "refnum out"=w526:T1)  [unwired: 4 in, 1 out]
                  n230 = call-poly <vilib>:"Read Key.vi"("section"=w534, "error in (no error)"=w527, "key"="Selected_Plot_0_0", "refnum"=w526) -> ("error out"=w547:errorcluster, "value"=w533:string, "refnum out"=w548:T1)  [unwired: 4 in, 1 out]
                  n231 = local write "select_plot_0"(w533) -> ()
                  n232 = call-poly <vilib>:"Read Key.vi"("section"=w534, "error in (no error)"=w547, "key"="Selected_Plot_0_1", "refnum"=w548) -> ("error out"=w544:errorcluster, "value"=w532:string, "refnum out"=w545:T1)  [unwired: 4 in, 1 out]
                  n233 = local write "select_plot_1"(w532) -> ()
                  n234 = call-poly <vilib>:"Read Key.vi"("section"=w534, "error in (no error)"=w544, "key"="Selected_Plot_0_2", "refnum"=w545) -> ("error out"=w541:errorcluster, "value"=w531:string, "refnum out"=w542:T1)  [unwired: 4 in, 1 out]
                  n235 = local write "select_plot_2"(w531) -> ()
                  n236 = call-poly <vilib>:"Read Key.vi"("section"=w534, "error in (no error)"=w541, "key"="Selected_Plot_0_3", "refnum"=w542) -> ("error out"=w538:errorcluster, "value"=w530:string, "refnum out"=w539:T1)  [unwired: 4 in, 1 out]
                  n237 = local write "select_plot_3"(w530) -> ()
                  n238 = call-poly <vilib>:"Read Key.vi"("section"=w534, "error in (no error)"=w538, "key"="Selected_Plot_0_4", "refnum"=w539) -> ("error out"=w536:errorcluster, "value"=w529:string, "refnum out"=w535:T1)  [unwired: 4 in, 1 out]
                  n239 = local write "select_plot_4"(w529) -> ()
                  n240 = call-poly <vilib>:"Read Key.vi"("section"=w534, "error in (no error)"=w536, "key"="Selected_Plot_0_5", "refnum"=w535) -> ("error out"=w521:errorcluster, "value"=w528:string, "refnum out"=w522:T1)  [unwired: 4 in, 1 out]
                  n241 = local write "enable_plot_5"(w575) -> ()
                  n242 = property on="color_picker_5" class="ColBox"("Val(Sgnl)"=w515) -> ()  [unwired: 2 in, 2 out]
                  n243 = local write "select_plot_5"(w528) -> ()
                  n244 = call <vilib>:"Close Config Data.vi"("error in (no error)"=w521, "refnum"=w522) -> ()  [unwired: 8 in, 2 out]
                  "loaded_config_path" <- w513
                }
              }
            }
          }
        }
        event "safe_config_plot_0": Value Change {
          n245 = event-data() -> ("NewVal"=w595:bool)  [unwired: 1 in, 5 out]
          n246 = case shown="True" w595 {
            selector: w595 -> [_ w601]
            tunnel: [_ w597] -> w594
            tunnel: [_ w596] -> w593
            frame False {
            }
            frame True {
              n247 = local read "loaded_config_filename"() -> (w598:string)
              n248 = Not(x=w601) -> (.not. x?=w602:bool)
              n249 = local write "safe_config_plot_0"(w602) -> ()
              n250 = Not Equal?(x=w598, y="") -> (x != y?=w599:bool)
              n251 = case shown="False" w599 {
                tunnel: w598 -> [_ w614]
                tunnel: [w604 w611] -> w597
                tunnel: [w605 w610] -> w596
                frame False {
                  n252 = call "File Dialog3"("pattern (all files)"="*.ini" ("pattern label"), "pattern label"="INI-File") -> ("selected path"=w605:path, "cancelled"=w606:bool, "error out"=w603:errorcluster)  [unwired: 10 in, 1 out]
                  n253 = Not(x=w606) -> (.not. x?=w604:bool)
                  n254 = call <vilib>:"Clear Errors.vi"("error in (no error)"=w603) -> ()  [unwired: 5 in, 2 out]
                }
                frame True {
                  n255 = local read "loaded_config_path"() -> (w610:path)
                  n256 = Concatenate Strings(w614, " will be overwritten!" ("string")) -> (w612:string)
                  n257 = call "Display Message to User"("Message"=w612) -> ("error out"=w609:errorcluster, "OK"=w611:bool)  [unwired: 9 in]
                  n258 = call <vilib>:"Clear Errors.vi"("error in (no error)"=w609) -> ()  [unwired: 5 in, 2 out]
                }
              }
            }
          }
        }
        event "safe_config_as_plot_0": Value Change {
          n259 = event-data() -> ("NewVal"=w617:bool)  [unwired: 1 in, 5 out]
          n260 = case shown="True" w617 {
            selector: w617 -> [_ w621]
            tunnel: [_ w620] -> w616
            tunnel: [_ w619] -> w615
            frame False {
            }
            frame True {
              n261 = Not(x=w621) -> (.not. x?=w622:bool)
              n262 = local write "safe_config_as_plot_0"(w622) -> ()
              n263 = call "File Dialog"("pattern (all files)"="*.ini" ("pattern label"), "pattern label"="INI-File") -> ("selected path"=w619:path, "cancelled"=w623:bool, "error out"=w618:errorcluster)  [unwired: 10 in, 1 out]
              n264 = Not(x=w623) -> (.not. x?=w620:bool)
              n265 = call <vilib>:"Clear Errors.vi"("error in (no error)"=w618) -> ()  [unwired: 5 in, 2 out]
            }
          }
        }
        event Timeout {
          n266 = event-data() -> ()  [unwired: 1 in, 3 out]
        }
      }
      n267 = case shown="True" w275 {
        tunnel: w274 -> [_ w279]
        frame False {
        }
        frame True {
          w286 = "Plot_Window" ("section")
          w331 = "Plot_Window" ("section")
          w280 = "Plot_Window" ("section")
          n268 = local read "color_picker_0"() -> (w338:u32)
          n269 = local read "enable_plot_0"() -> (w326:bool)
          n270 = local read "select_plot_0"() -> (w291:string)
          n271 = Build Path(name or relative path=w279) -> (appended path=w344:path)  [unwired: 1 in]
          n272 = call <vilib>:"Open Config Data.vi"("configuration file path"=w344) -> ("error out"=w343:errorcluster, "refnum"=w342:T1)  [unwired: 8 in, 1 out]
          n273 = call-poly <vilib>:"Write Key.vi"("section"=w280, "error in (no error)"=w343, "value"=w338, "key"="Color_Plot_0_0", "refnum"=w342) -> ("error out"=w354:errorcluster, "refnum out"=w355:T1)  [unwired: 4 in, 1 out]
          n274 = local read "enable_plot_1"() -> (w327:bool)
          n275 = local read "color_picker_1"() -> (w337:u32)
          n276 = local read "select_plot_1"() -> (w290:string)
          n277 = call-poly <vilib>:"Write Key.vi"("section"=w280, "error in (no error)"=w354, "value"=w337, "key"="Color_Plot_0_1", "refnum"=w355) -> ("error out"=w351:errorcluster, "refnum out"=w352:T1)  [unwired: 4 in, 1 out]
          n278 = local read "enable_plot_2"() -> (w328:bool)
          n279 = local read "color_picker_2"() -> (w336:u32)
          n280 = local read "select_plot_2"() -> (w289:string)
          n281 = call-poly <vilib>:"Write Key.vi"("section"=w280, "error in (no error)"=w351, "value"=w336, "key"="Color_Plot_0_2", "refnum"=w352) -> ("error out"=w348:errorcluster, "refnum out"=w349:T1)  [unwired: 4 in, 1 out]
          n282 = local read "color_picker_3"() -> (w333:u32)
          n283 = local read "enable_plot_3"() -> (w332:bool)
          n284 = local read "select_plot_3"() -> (w285:string)
          n285 = call-poly <vilib>:"Write Key.vi"("section"=w280, "error in (no error)"=w348, "value"=w333, "key"="Color_Plot_0_3", "refnum"=w349) -> ("error out"=w345:errorcluster, "refnum out"=w346:T1)  [unwired: 4 in, 1 out]
          n286 = local read "color_picker_4"() -> (w335:u32)
          n287 = local read "enable_plot_4"() -> (w329:bool)
          n288 = local read "select_plot_4"() -> (w288:string)
          n289 = call-poly <vilib>:"Write Key.vi"("section"=w280, "error in (no error)"=w345, "value"=w335, "key"="Color_Plot_0_4", "refnum"=w346) -> ("error out"=w339:errorcluster, "refnum out"=w340:T1)  [unwired: 4 in, 1 out]
          n290 = local read "color_picker_5"() -> (w334:u32)
          n291 = local read "enable_plot_5"() -> (w330:bool)
          n292 = local read "select_plot_5"() -> (w287:string)
          n293 = call-poly <vilib>:"Write Key.vi"("section"=w280, "error in (no error)"=w339, "value"=w334, "key"="Color_Plot_0_5", "refnum"=w340) -> ("error out"=w309:errorcluster, "refnum out"=w308:T1)  [unwired: 4 in, 1 out]
          n294 = call-poly <vilib>:"Write Key.vi"("section"=w331, "error in (no error)"=w309, "value"=w326, "key"="Enable_Plot_0_0", "refnum"=w308) -> ("error out"=w313:errorcluster, "refnum out"=w312:T1)  [unwired: 4 in, 1 out]
          n295 = call-poly <vilib>:"Write Key.vi"("section"=w331, "error in (no error)"=w313, "value"=w327, "key"="Enable_Plot_0_1", "refnum"=w312) -> ("error out"=w316:errorcluster, "refnum out"=w315:T1)  [unwired: 4 in, 1 out]
          n296 = call-poly <vilib>:"Write Key.vi"("section"=w331, "error in (no error)"=w316, "value"=w328, "key"="Enable_Plot_0_2", "refnum"=w315) -> ("error out"=w319:errorcluster, "refnum out"=w318:T1)  [unwired: 4 in, 1 out]
          n297 = call-poly <vilib>:"Write Key.vi"("section"=w331, "error in (no error)"=w319, "value"=w332, "key"="Enable_Plot_0_3", "refnum"=w318) -> ("error out"=w322:errorcluster, "refnum out"=w321:T1)  [unwired: 4 in, 1 out]
          n298 = call-poly <vilib>:"Write Key.vi"("section"=w331, "error in (no error)"=w322, "value"=w329, "key"="Enable_Plot_0_4", "refnum"=w321) -> ("error out"=w325:errorcluster, "refnum out"=w324:T1)  [unwired: 4 in, 1 out]
          n299 = call-poly <vilib>:"Write Key.vi"("section"=w331, "error in (no error)"=w325, "value"=w330, "key"="Enable_Plot_0_5", "refnum"=w324) -> ("error out"=w284:errorcluster, "refnum out"=w283:T1)  [unwired: 4 in, 1 out]
          n300 = call-poly <vilib>:"Write Key.vi"("section"=w286, "error in (no error)"=w284, "value"=w291, "key"="Selected_Plot_0_0", "refnum"=w283) -> ("error out"=w304:errorcluster, "refnum out"=w305:T1)  [unwired: 4 in, 1 out]
          n301 = call-poly <vilib>:"Write Key.vi"("section"=w286, "error in (no error)"=w304, "value"=w290, "key"="Selected_Plot_0_1", "refnum"=w305) -> ("error out"=w301:errorcluster, "refnum out"=w302:T1)  [unwired: 4 in, 1 out]
          n302 = call-poly <vilib>:"Write Key.vi"("section"=w286, "error in (no error)"=w301, "value"=w289, "key"="Selected_Plot_0_2", "refnum"=w302) -> ("error out"=w298:errorcluster, "refnum out"=w299:T1)  [unwired: 4 in, 1 out]
          n303 = call-poly <vilib>:"Write Key.vi"("section"=w286, "error in (no error)"=w298, "value"=w285, "key"="Selected_Plot_0_3", "refnum"=w299) -> ("error out"=w295:errorcluster, "refnum out"=w296:T1)  [unwired: 4 in, 1 out]
          n304 = call-poly <vilib>:"Write Key.vi"("section"=w286, "error in (no error)"=w295, "value"=w288, "key"="Selected_Plot_0_4", "refnum"=w296) -> ("error out"=w292:errorcluster, "refnum out"=w293:T1)  [unwired: 4 in, 1 out]
          n305 = call-poly <vilib>:"Write Key.vi"("section"=w286, "error in (no error)"=w292, "value"=w287, "key"="Selected_Plot_0_5", "refnum"=w293) -> ("error out"=w281:errorcluster, "refnum out"=w282:T1)  [unwired: 4 in, 1 out]
          n306 = call <vilib>:"Close Config Data.vi"("error in (no error)"=w281, "refnum"=w282) -> ()  [unwired: 8 in, 2 out]
        }
      }
      n307 = case shown="True" w276 {
        frame False {
        }
        frame True {
          n308 = call "fgv_cursor_data.vi"() -> ("cursor_idx_get"=w386:i32, "cursor_data_get"=w358:T7)  [unwired: 9 in, 5 out]
          n309 = Unbundle(w358) -> ("cursor_data"=w385:dbl[], "frequency"=w384:string, "wavelength_m"=w383:dbl)
          n310 = Index Array(array=w385) -> (element #1=w374:dbl, element #2=w376:dbl, element #3=w378:dbl, element #4=w379:dbl, element #5=w364:dbl, element #6=w363:dbl)  [unwired: 6 in]
          n311 = local read "select_plot_0"() -> (w367:string)
          n312 = local read "select_plot_1"() -> (w368:string)
          n313 = local read "select_plot_2"() -> (w369:string)
          n314 = local read "select_plot_3"() -> (w380:string)
          n315 = local read "select_plot_4"() -> (w366:string)
          n316 = local read "select_plot_5"() -> (w365:string)
          n317 = call "get_plot_y_scale_data.vi"("plot_selector"=w367, "cursor_value_in"=w374) -> ("prefix/unit"=w372:string, "cursor_value_out"=w373:dbl)  [unwired: 8 in]
          n318 = call "get_plot_y_scale_data.vi"("plot_selector"=w368, "cursor_value_in"=w376) -> ("prefix/unit"=w371:string, "cursor_value_out"=w375:dbl)  [unwired: 8 in]
          n319 = call "get_plot_y_scale_data.vi"("plot_selector"=w369, "cursor_value_in"=w378) -> ("prefix/unit"=w370:string, "cursor_value_out"=w377:dbl)  [unwired: 8 in]
          n320 = call "get_plot_y_scale_data.vi"("plot_selector"=w380, "cursor_value_in"=w379) -> ("prefix/unit"=w382:string, "cursor_value_out"=w381:dbl)  [unwired: 8 in]
          n321 = call "get_plot_y_scale_data.vi"("plot_selector"=w366, "cursor_value_in"=w364) -> ("prefix/unit"=w362:string, "cursor_value_out"=w361:dbl)  [unwired: 8 in]
          n322 = call "get_plot_y_scale_data.vi"("plot_selector"=w365, "cursor_value_in"=w363) -> ("prefix/unit"=w360:string, "cursor_value_out"=w359:dbl)  [unwired: 8 in]
          n323 = case shown="0, Default" w386 {
            tunnel: w373 -> [w400 w414]
            tunnel: w375 -> [w399 w412]
            tunnel: w377 -> [w398 w410]
            tunnel: w381 -> [w397 w408]
            tunnel: w384 -> [w396 w406]
            tunnel: w383 -> [w395 w405]
            tunnel: w382 -> [w394 w407]
            tunnel: w372 -> [w393 w413]
            tunnel: w371 -> [w392 w411]
            tunnel: w370 -> [w391 w409]
            tunnel: w362 -> [w390 w403]
            tunnel: w361 -> [w389 w404]
            tunnel: w360 -> [w388 w401]
            tunnel: w359 -> [w387 w402]
            frame 0, Default {
              n324 = local write "cursor_p0_1"(w400) -> ()
              n325 = local write "cursor_p0_1_prefix"(w393) -> ()
              n326 = local write "cursor_p1_1"(w399) -> ()
              n327 = local write "cursor_p1_1_prefix"(w392) -> ()
              n328 = local write "cursor_p2_1"(w398) -> ()
              n329 = local write "cursor_p2_1_prefix"(w391) -> ()
              n330 = local write "cursor_p3_1"(w397) -> ()
              n331 = local write "cursor_p3_1_prefix"(w394) -> ()
              n332 = local write "cursor_p0_freq_1"(w396) -> ()
              n333 = local write "cursor_p0_wavel_1"(w395) -> ()
              n334 = local write "cursor_p4_1"(w389) -> ()
              n335 = local write "cursor_p4_1_prefix"(w390) -> ()
              n336 = local write "cursor_p5_1"(w387) -> ()
              n337 = local write "cursor_p5_1_prefix"(w388) -> ()
            }
            frame 1 {
              n338 = local write "cursor_p0_2"(w414) -> ()
              n339 = local write "cursor_p0_2_prefix"(w413) -> ()
              n340 = local write "cursor_p1_2"(w412) -> ()
              n341 = local write "cursor_p1_2_prefix"(w411) -> ()
              n342 = local write "cursor_p2_2"(w410) -> ()
              n343 = local write "cursor_p2_2_prefix"(w409) -> ()
              n344 = local write "cursor_p3_2"(w408) -> ()
              n345 = local write "cursor_p3_2_prefix"(w407) -> ()
              n346 = local write "cursor_p0_freq_2"(w406) -> ()
              n347 = local write "cursor_p0_wavel_2"(w405) -> ()
              n348 = local write "cursor_p4_2"(w404) -> ()
              n349 = local write "cursor_p4_2_prefix"(w403) -> ()
              n350 = local write "cursor_p5_2"(w402) -> ()
              n351 = local write "cursor_p5_2_prefix"(w401) -> ()
            }
          }
        }
      }
    }
    n352 = call "Is Value Changed.vim"("value"="enable_plot_2") -> ("changed or first call?"=w46:bool)
    n353 = call "Is Value Changed.vim"("value"="enable_plot_0") -> ("changed or first call?"=w29:bool)
    n354 = case shown="True" w46 {
      tunnel: "enable_plot_2" -> [_ w262]
      tunnel: w44 -> [_ w265]
      tunnel: 2 ("plot_id") -> [_ w264]
      frame False {
      }
      frame True {
        n355 = property on="Property Node" class="XYGraph (strict)" props=["Active Plot", "Plot", "Visible?", "Plot", "YScaleIdx"](reference=w265, "Active Plot"=w264, "Plot.Visible?"=w262) -> (reference out=w263:refnum<vi>)  [unwired: 1 in, 2 out]
        n356 = call "show_plot_y_axis.vi"("plot_ref_in"=w263) -> ()  [unwired: 9 in, 2 out]
      }
    }
    n357 = case shown="True" w29 {
      tunnel: "enable_plot_0" -> [_ w271]
      tunnel: w44 -> [_ w273]
      tunnel: 0 ("plot_id") -> [_ w272]
      frame False {
      }
      frame True {
        n358 = property on="Property Node" class="XYGraph (strict)" props=["Active Plot", "Plot", "Visible?", "Plot", "YScaleIdx"](reference=w273, "Active Plot"=w272, "Plot.Visible?"=w271) -> (reference out=w270:refnum<vi>)  [unwired: 1 in, 2 out]
        n359 = call "show_plot_y_axis.vi"("plot_ref_in"=w270) -> ()  [unwired: 9 in, 2 out]
      }
    }
    n360 = control-ref of="plot_0"() -> (w34:refnum<vi>)
    n361 = call "Is Value Changed.vim"("value"="enable_plot_1") -> ("changed or first call?"=w49:bool)
    n362 = call "Is Value Changed.vim"("value"="enable_plot_3") -> ("changed or first call?"=w32:bool)
    n363 = case shown="True" w32 {
      tunnel: "enable_plot_3" -> [_ w234]
      tunnel: w34 -> [_ w237]
      tunnel: 3 ("plot_id") -> [_ w236]
      frame False {
      }
      frame True {
        n364 = property on="Property Node" class="XYGraph (strict)" props=["Active Plot", "Plot", "Visible?", "Plot", "YScaleIdx"](reference=w237, "Active Plot"=w236, "Plot.Visible?"=w234) -> (reference out=w235:refnum<vi>)  [unwired: 1 in, 2 out]
        n365 = call "show_plot_y_axis.vi"("plot_ref_in"=w235) -> ()  [unwired: 9 in, 2 out]
      }
    }
    n366 = case shown="True" w49 {
      tunnel: "enable_plot_1" -> [_ w266]
      tunnel: w34 -> [_ w269]
      tunnel: 1 ("plot_id") -> [_ w268]
      frame False {
      }
      frame True {
        n367 = property on="Property Node" class="XYGraph (strict)" props=["Active Plot", "Plot", "Visible?", "Plot", "YScaleIdx"](reference=w269, "Active Plot"=w268, "Plot.Visible?"=w266) -> (reference out=w267:refnum<vi>)  [unwired: 1 in, 2 out]
        n368 = call "show_plot_y_axis.vi"("plot_ref_in"=w267) -> ()  [unwired: 9 in, 2 out]
      }
    }
    n369 = control-ref of="plot_0"() -> (w19:refnum<vi>)
    n370 = call "Is Value Changed.vim"("value"="enable_plot_5") -> ("changed or first call?"=w21:bool)
    n371 = call "Is Value Changed.vim"("value"="enable_plot_4") -> ("changed or first call?"=w24:bool)
    n372 = case shown="True" w21 {
      tunnel: "enable_plot_5" -> [_ w225]
      tunnel: w19 -> [_ w228]
      tunnel: 5 ("plot_id") -> [_ w227]
      frame False {
      }
      frame True {
        n373 = property on="Property Node" class="XYGraph (strict)" props=["Active Plot", "Plot", "Visible?", "Plot", "YScaleIdx"](reference=w228, "Active Plot"=w227, "Plot.Visible?"=w225) -> (reference out=w226:refnum<vi>)  [unwired: 1 in, 2 out]
        n374 = call "show_plot_y_axis.vi"("plot_ref_in"=w226) -> ()  [unwired: 9 in, 2 out]
      }
    }
    n375 = case shown="True" w24 {
      tunnel: "enable_plot_4" -> [_ w229]
      tunnel: w19 -> [_ w232]
      tunnel: 4 ("plot_id") -> [_ w231]
      frame False {
      }
      frame True {
        n376 = property on="Property Node" class="XYGraph (strict)" props=["Active Plot", "Plot", "Visible?", "Plot", "YScaleIdx"](reference=w232, "Active Plot"=w231, "Plot.Visible?"=w229) -> (reference out=w230:refnum<vi>)  [unwired: 1 in, 2 out]
        n377 = call "show_plot_y_axis.vi"("plot_ref_in"=w230) -> ()  [unwired: 9 in, 2 out]
      }
    }
    n378 = call "fgv_cursor_data.vi"() -> ("cursor_idx_get"=w12:i32, "cursor_pos_get"=w10:i32, "cursor_color_get"=w5:T8, "plot_id_get"=w11:i32, "cursor_mode_get"=w7:bool)  [unwired: 9 in, 2 out]
    n379 = call "Is Value Changed.vim"("value"=w5) -> ("changed or first call?"=w6:bool)
    n380 = call "Is Value Changed.vim"("value"=w10) -> ("changed or first call?"=w8:bool)
    n381 = And(x=w8, y=w7) -> (x .and. y?=w9:bool)
    n382 = case shown="True" w6 {
      tunnel: w5 -> [_ w56]
      frame False {
      }
      frame True {
        n383 = Unbundle(w56) -> ("cursor_0_color"=w52:u32, "cursor_1_color"=w53:u32)
        n384 = property on="plot_0" class="XYGraph (strict)"("Active Cursor"=u32 0, "Cursor.Cursor Color"=w52) -> ()  [unwired: 2 in, 2 out]
        n385 = property on="plot_0" class="XYGraph (strict)"("Active Cursor"=u32 1, "Cursor.Cursor Color"=w53) -> ()  [unwired: 2 in, 2 out]
      }
    }
    n386 = case shown="True" w9 {
      tunnel: w10 -> [_ w59]
      tunnel: w12 -> [_ w58]
      tunnel: w11 -> [_ w57]
      frame False {
      }
      frame True {
        n387 = case shown="99, Default" w57 {
          tunnel: w58 -> [_ w63]
          tunnel: w59 -> [_ w62]
          frame 10 {
          }
          frame 99, Default {
            n388 = property on="plot_0" class="XYGraph (strict)"("Active Cursor"=w63, "Cursor.Cursor Index"=w62) -> (error out=w60:errorcluster, "Value"=w61:cluster{"array type (2D Dbl)":dbl[], dbl[]}[])  [unwired: 2 in, 1 out]
            n389 = property on="plot_0" class="XYGraph (strict)"(error in=w60, "Val(Sgnl)"=w61) -> ()  [unwired: 1 in, 2 out]
          }
        }
      }
    }
    n390 = Wait (ms)(milliseconds to wait=u32 15) -> ()  [unwired: 1 out]
  }
  n391 = Release Notifier(notifier=w1) -> ()  [unwired: 2 in, 3 out]
